vi "Tango.vi"(9 "Stage Action":T1={"Action"=enum."Get Position", "Axis"=[], "Setpoint"=[], "Velocity"=0.5, "Cmd Recvd?"=FALSE, "Position"=[], "Status"=enum."Error", "Misc"=variant} {"Velocity" min=0.0 max=1.0 step=0.01}, 10 "Scan IM Notifier":refnum<notifier>, 11 "Tango Handle":i32) -> (3 "Tango Handle":i32)   [LabVIEW 2016]
uses:
  Stages Controls/Stage Notifier Element.ctl
  Stages Controls/Stage Actions.ctl
  Stages Controls/Stage Status.ctl
  <userlib>/Tango_DLL/Tango_DLL.lvlib
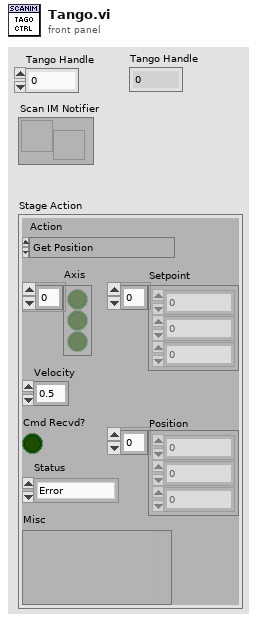
[diagram p1: front panel]
types:
  T1 = typedef "Stage Notifier Element.ctl" = cluster{"Action":T2, "Axis":bool[], "Setpoint":dbl[], "Velocity":dbl, "Cmd Recvd?":bool, "Position":dbl[], "Status":T3, "Misc":variant}
  T2 = typedef "Stage Actions.ctl" = enum16{"Get Position", "MVR", "MOVE", "HALT", "ONTARGET", "ERROR", "REFERENCE", "INIT", "VELOCITY", "STATUS", "EXIT", "HOME", "ZEROPOS", "NANOPOS", "ANALOG", "QUIT"}
  T3 = typedef "Stage Status.ctl" = enum16{"Error", "Abort", "Busy", "On Target"}
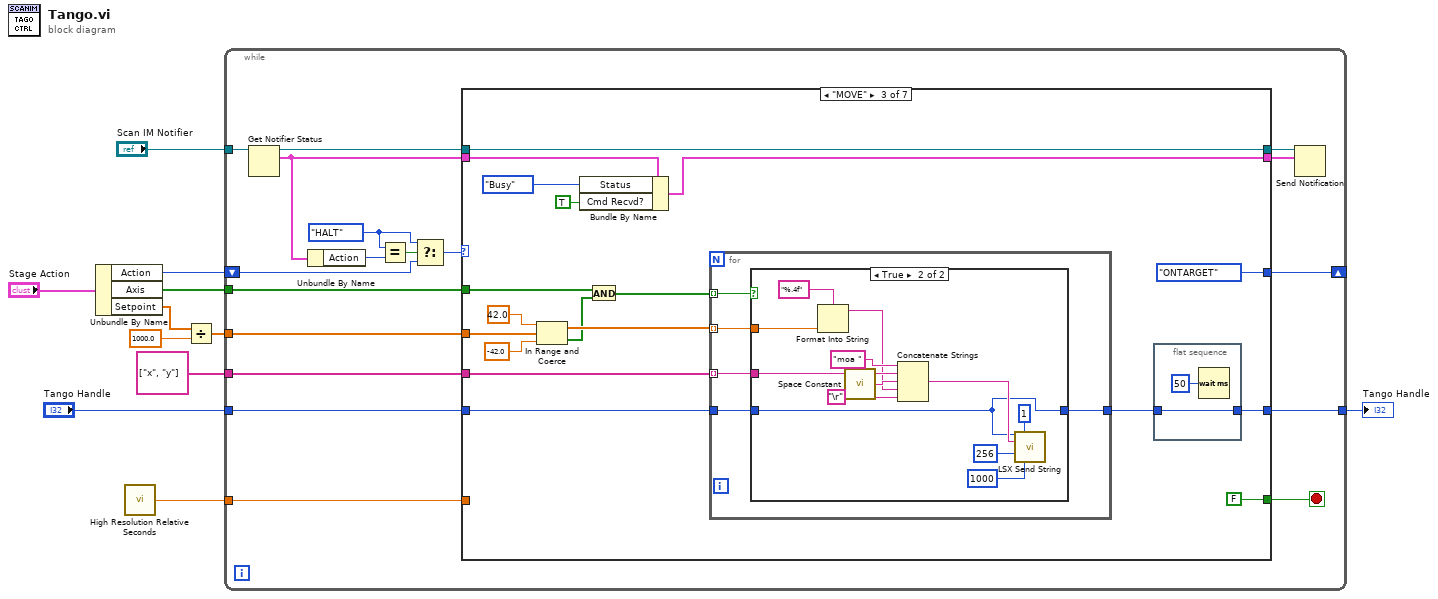
[diagram p0: block diagram]
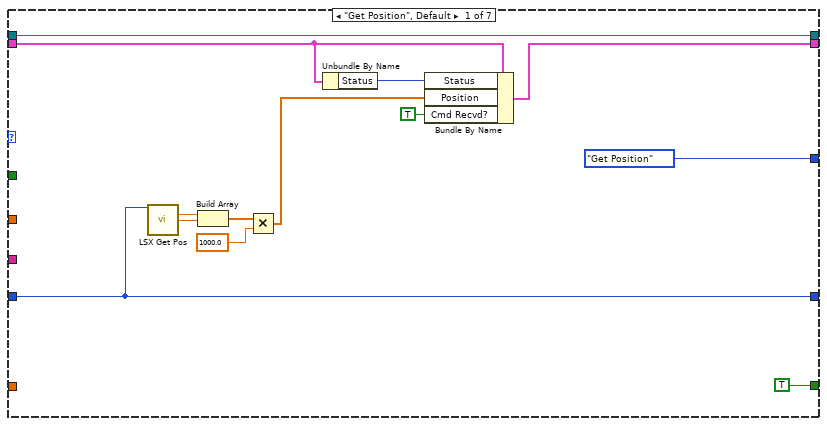
[diagram p2: hidden frame]
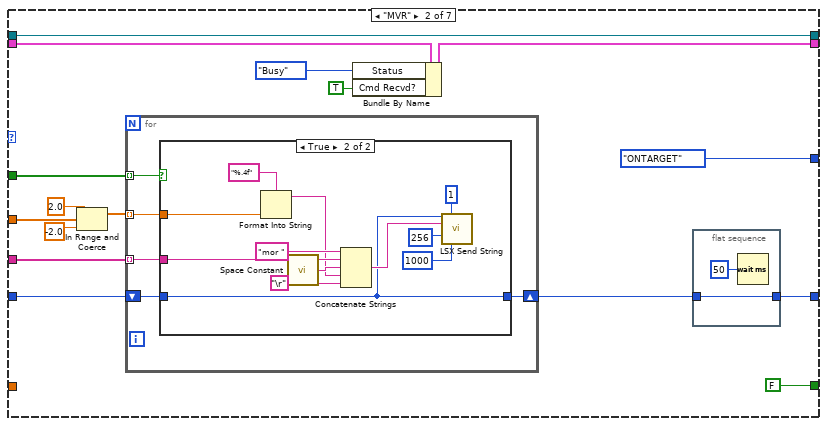
[diagram p3: hidden frame]
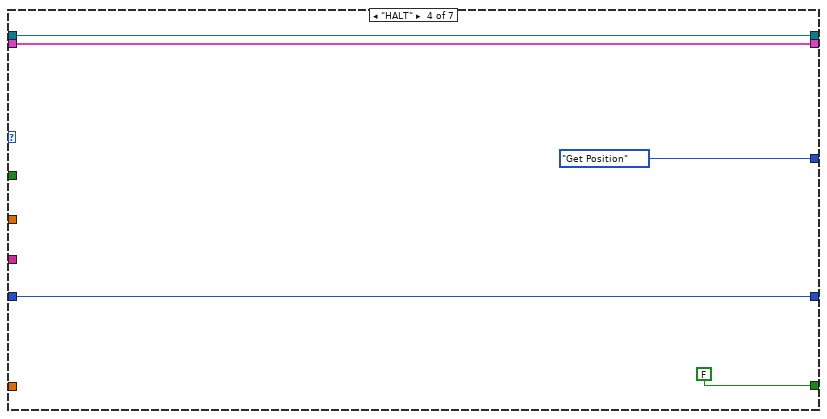
[diagram p6: hidden frame]
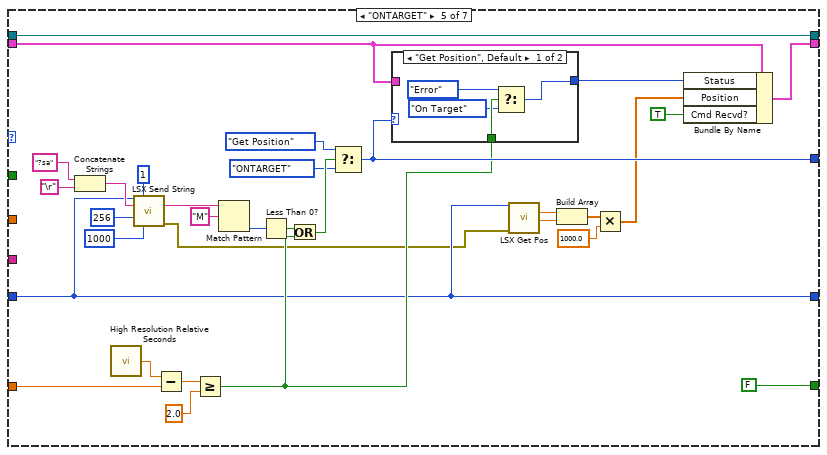
[diagram p7: hidden frame]
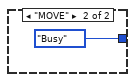
[diagram p8: hidden frame]
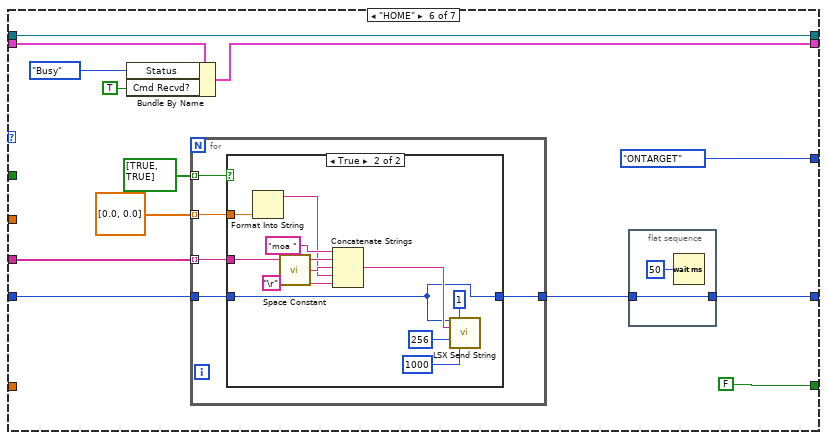
[diagram p9: hidden frame]
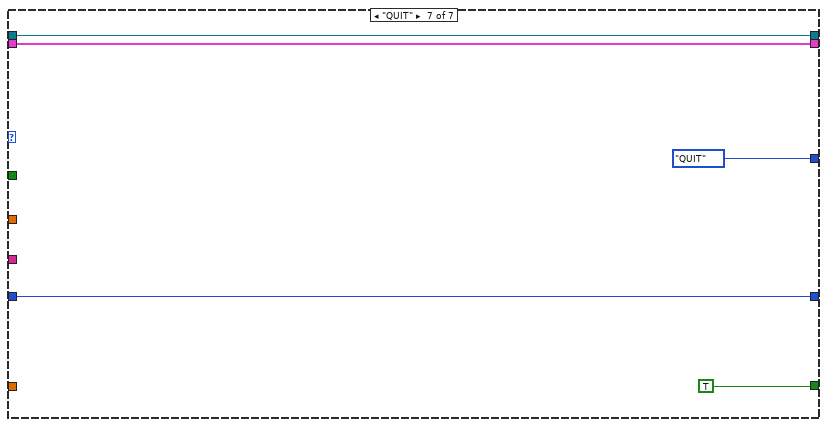
[diagram p11: hidden frame]
diagram:
  n1 = Unbundle By Name("Stage Action") -> ("Action"=w5:T2, "Axis"=w8:bool[], "Setpoint"=w3:dbl[])
  n2 = call <vilib>:"High Resolution Relative Seconds.vi"() -> ("relative seconds"=w7:dbl)
  n3 = Divide(x=w3, y=1000.0) -> (x/y=w1:dbl[])
  n4 = while {
    shift-right: [w27] -> _
    shift-left: w5 -> [w15]
    tunnel: "Tango Handle" -> [w28]
    tunnel: [w26] -> w11
    tunnel: w8 -> [w25]
    tunnel: "Scan IM Notifier" -> [w21]
    tunnel: w7 -> [w19]
    tunnel: w1 -> [w24]
    tunnel: string[] ["x", "y"] -> [w12]
    stop <- w29 stop-if-true
    w13 = Stage_Actions."HALT" ("x")
    n5 = Get Notifier Status(notifier=w21) -> (notifier out=w20:refnum<notifier>, current notification=w17:T1)  [unwired: 1 in, 3 out]
    n6 = Unbundle By Name(w17) -> ("Action"=w18:T2)
    n7 = Equal?(x=w13, y=w18) -> (x = y?=w16:bool)
    n8 = Select(t=w13, s=w16, f=w15) -> (s? t:f=w14:T2)
    n9 = case shown="\"MOVE\"" w14 {
      tunnel: [TRUE FALSE FALSE FALSE FALSE FALSE TRUE] -> w29
      tunnel: w28 -> [w32 w58 w96 w121 w126 w171 w191]
      tunnel: [Stage_Actions."Get Position" ("x") Stage_Actions."ONTARGET" ("x") Stage_Actions."ONTARGET" ("x") Stage_Actions."Get Position" ("x") w149 Stage_Actions."ONTARGET" ("x") Stage_Actions."QUIT" ("x")] -> w27
      tunnel: [w32 w52 w91 w121 w126 w170 w191] -> w26
      tunnel: w25 -> [_ w57 w80 _ _ _ _]
      tunnel: w24 -> [_ w54 w93 _ _ _ _]
      tunnel: w20 -> [w39 w47 w86 w119 w148 w165 w194]
      tunnel: [w39 w47 w86 w119 w148 w165 w194] -> w23
      tunnel: [w40 w48 w87 w118 w152 w166 w193] -> w22
      tunnel: w17 -> [w38 w46 w85 w118 w150 w164 w193]
      tunnel: w19 -> [_ _ _ _ w151 _ _]
      tunnel: w12 -> [_ w43 w82 _ _ w161 _]
      frame "Get Position", Default {
        n10 = call <userlib>:"LSX Get Pos.vi"("lLSID"=w32) -> ("pdX out"=w34:dbl, "pdY out"=w33:dbl)  [unwired: 9 in, 4 out]
        n11 = Build Array(w34, w33) -> (w36:dbl[])
        n12 = Multiply(x=w36, y=1000.0) -> (x*y=w31:dbl[])
        n13 = Unbundle By Name(w38) -> ("Status"=w37:T3)
        n14 = Bundle By Name(cluster=w38, "Status"=w37, "Position"=w31, "Cmd Recvd?"=TRUE) -> (w40:T1)
      }
      frame "MVR" {
        n15 = In Range and Coerce(upper limit=2.0, x=w54, lower limit=-2.0) -> (coerced(x)=w53:dbl[])  [unwired: 1 out]
        n16 = for {
          shift-right: [w64] -> w51
          shift-left: w58 -> [w65]
          tunnel: w57 -> [w63] mode=indexing
          tunnel: w53 -> [w62] mode=indexing
          tunnel: w43 -> [w61] mode=indexing
          n17 = case shown="True" w63 {
            tunnel: w65 -> [w66 w68]
            tunnel: [w66 w68] -> w64
            tunnel: w62 -> [_ w76]
            tunnel: w61 -> [_ w74]
            frame False {
            }
            frame True {
              n18 = Format Into String(format string="%.4f", w76) -> (resulting string=w72:string)  [unwired: 2 in, 1 out]
              n19 = call <vilib>:"Space Constant.vi"() -> ("String"=w73:string)
              n20 = Concatenate Strings("mor ", w74, w73, w72, "\r") -> (w71:string)
              n21 = call <userlib>:"LSX Send String.vi"("lLSID"=w68, "bReadLine"=1, "pcStr"=w71, "lMaxLen"=256, "lTimeOut"=1000) -> ()  [unwired: 7 in, 4 out]
            }
          }
        }
        n22 = Bundle By Name(cluster=w46, "Status"=Stage_Status."Busy", "Cmd Recvd?"=TRUE) -> (w48:T1)
        n23 = flat-sequence {
          tunnel: [w60] -> w52
          tunnel: w51 -> [w60]
          frame #0 {
            n24 = Wait (ms)(milliseconds to wait=u32 50) -> ()  [unwired: 1 out]
          }
        }
      }
      frame "MOVE" {
        n25 = In Range and Coerce(upper limit=42.0, x=w93, lower limit=-42.0) -> (coerced(x)=w92:dbl[], In Range?=w81:bool[])
        n26 = Bundle By Name(cluster=w85, "Status"=Stage_Status."Busy", "Cmd Recvd?"=TRUE) -> (w87:T1)
        n27 = And(x=w80, y=w81) -> (x .and. y?=w79:bool[])
        n28 = for {
          tunnel: w79 -> [w101] mode=indexing
          tunnel: w92 -> [w100] mode=indexing
          tunnel: w82 -> [w99] mode=indexing
          tunnel: w96 -> [w103]
          tunnel: [w102] -> w90
          n29 = case shown="True" w101 {
            tunnel: w103 -> [w104 w106]
            tunnel: [w104 w106] -> w102
            tunnel: w100 -> [_ w114]
            tunnel: w99 -> [_ w112]
            frame False {
            }
            frame True {
              n30 = Format Into String(format string="%.4f", w114) -> (resulting string=w110:string)  [unwired: 2 in, 1 out]
              n31 = call <vilib>:"Space Constant.vi"() -> ("String"=w111:string)
              n32 = Concatenate Strings("moa ", w112, w111, w110, "\r") -> (w109:string)
              n33 = call <userlib>:"LSX Send String.vi"("lLSID"=w106, "bReadLine"=1, "pcStr"=w109, "lMaxLen"=256, "lTimeOut"=1000) -> ()  [unwired: 7 in, 4 out]
            }
          }
        }
        n34 = flat-sequence {
          tunnel: [w98] -> w91
          tunnel: w90 -> [w98]
          frame #0 {
            n35 = Wait (ms)(milliseconds to wait=u32 50) -> ()  [unwired: 1 out]
          }
        }
      }
      frame "HALT" {
      }
      frame "ONTARGET" {
        n36 = Concatenate Strings("?sa" ("pcStr"), "\r") -> (w133:string)
        n37 = call <vilib>:"High Resolution Relative Seconds.vi"() -> ("relative seconds"=w145:dbl)
        n38 = call <userlib>:"LSX Send String.vi"("lLSID"=w126, "bReadLine"=1, "pcStr"=w133, "lMaxLen"=256, "lTimeOut"=1000) -> ("pcStr out"=w132:string, "error out"=w123:errorcluster)  [unwired: 7 in, 2 out]
        n39 = Subtract(x=w145, y=w151) -> (x-y=w144:dbl)
        n40 = Greater Or Equal?(x=w144, y=2.0) -> (x >= y?=w142:bool)
        n41 = Match Pattern(string=w132, regular expression="M") -> (offset past match=w130:i32)  [unwired: 1 in, 3 out]
        n42 = Less Than 0?(x=w130) -> (x < 0?=w129:bool)
        n43 = Or(x=w129, y=w142) -> (x .or. y?=w147:bool)
        n44 = Select(t=Stage_Actions."Get Position" ("x"), s=w147, f=Stage_Actions."ONTARGET" ("x")) -> (s? t:f=w149:T2)
        n45 = case shown="\"Get Position\", Default" w149 {
          tunnel: w150 -> [_ _]
          tunnel: [w156 Stage_Status."Busy" ("Status")] -> w139
          tunnel: w142 -> [w157 _]
          frame "Get Position", Default {
            n46 = Select(t=Stage_Status."Error" ("Status"), s=w157, f=Stage_Status."On Target" ("Status")) -> (s? t:f=w156:T3)
          }
          frame "MOVE" {
          }
        }
        n47 = call <userlib>:"LSX Get Pos.vi"("lLSID"=w126, "error in (no error)"=w123) -> ("pdX out"=w128:dbl, "pdY out"=w127:dbl)  [unwired: 8 in, 4 out]
        n48 = Build Array(w128, w127) -> (w125:dbl[])
        n49 = Multiply(x=w125, y=1000.0) -> (x*y=w122:dbl[])
        n50 = Bundle By Name(cluster=w150, "Status"=w139, "Position"=w122, "Cmd Recvd?"=TRUE) -> (w152:T1)
      }
      frame "HOME" {
        n51 = Bundle By Name(cluster=w164, "Status"=Stage_Status."Busy", "Cmd Recvd?"=TRUE) -> (w166:T1)
        n52 = for {
          tunnel: bool[] [TRUE, TRUE] -> [w176] mode=indexing
          tunnel: dbl[] [0.0, 0.0] -> [w175] mode=indexing
          tunnel: w161 -> [w174] mode=indexing
          tunnel: w171 -> [w178]
          tunnel: [w177] -> w169
          n53 = case shown="True" w176 {
            tunnel: w178 -> [w179 w180]
            tunnel: [w179 w180] -> w177
            tunnel: w175 -> [_ w188]
            tunnel: w174 -> [_ w186]
            frame False {
            }
            frame True {
              n54 = Format Into String(w188) -> (resulting string=w184:string)  [unwired: 3 in, 1 out]
              n55 = call <vilib>:"Space Constant.vi"() -> ("String"=w185:string)
              n56 = Concatenate Strings("moa ", w186, w185, w184, "\r") -> (w183:string)
              n57 = call <userlib>:"LSX Send String.vi"("lLSID"=w180, "bReadLine"=1, "pcStr"=w183, "lMaxLen"=256, "lTimeOut"=1000) -> ()  [unwired: 7 in, 4 out]
            }
          }
        }
        n58 = flat-sequence {
          tunnel: [w173] -> w170
          tunnel: w169 -> [w173]
          frame #0 {
            n59 = Wait (ms)(milliseconds to wait=u32 50) -> ()  [unwired: 1 out]
          }
        }
      }
      frame "QUIT" {
      }
    }
    n60 = Send Notification(notification=w22, notifier=w23) -> ()  [unwired: 1 in, 2 out]
  }
  "Tango Handle" <- w11
